vi "query UL_DL Center Channel Number.vi"(8 "error in (no error)":errorcluster, 9 "Direction":T2, 10 "Selected CC Argements":T1, 11 "NR in":refnum<class "NR.lvclass">) -> (0 "error out":errorcluster, 2 "Center Channel Number":u32, 3 "NR out":refnum<class "NR.lvclass">)   [LabVIEW 2023, in "ANRITSU Call Box.lvlib" / "NR.lvclass"]
uses:
  NR.lvclass
  NR.lvclass/NR.ctl
  Type Definition/Uplink Downlink Enum.ctl
  ANRITSU Call Box.lvlib
  Type Definition/NR Selected CC Type Arguments.ctl
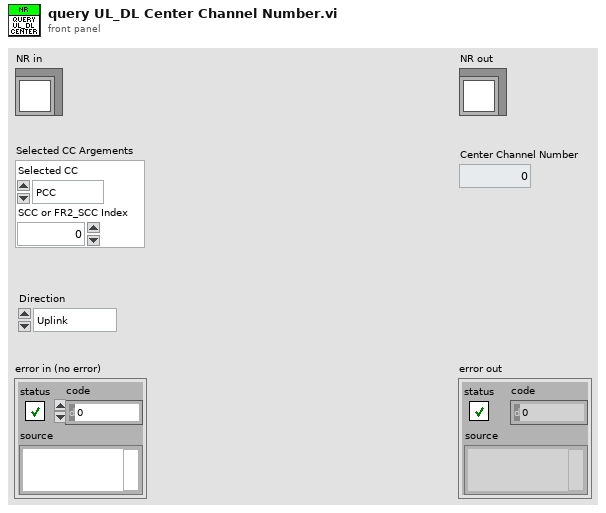
[diagram p1: front panel]
types:
  T1 = typedef "ANRITSU Call Box.lvlib/NR Selected CC Type Arguments.ctl" = cluster{"Selected CC":enum16{"PCC", "SCC", "FR2_PCC", "FR2_SCC"}, "SCC or FR2_SCC Index":u32}
  T2 = typedef "ANRITSU Call Box.lvlib/Uplink Downlink Enum.ctl" = enum16{"Uplink", "Downlink"}
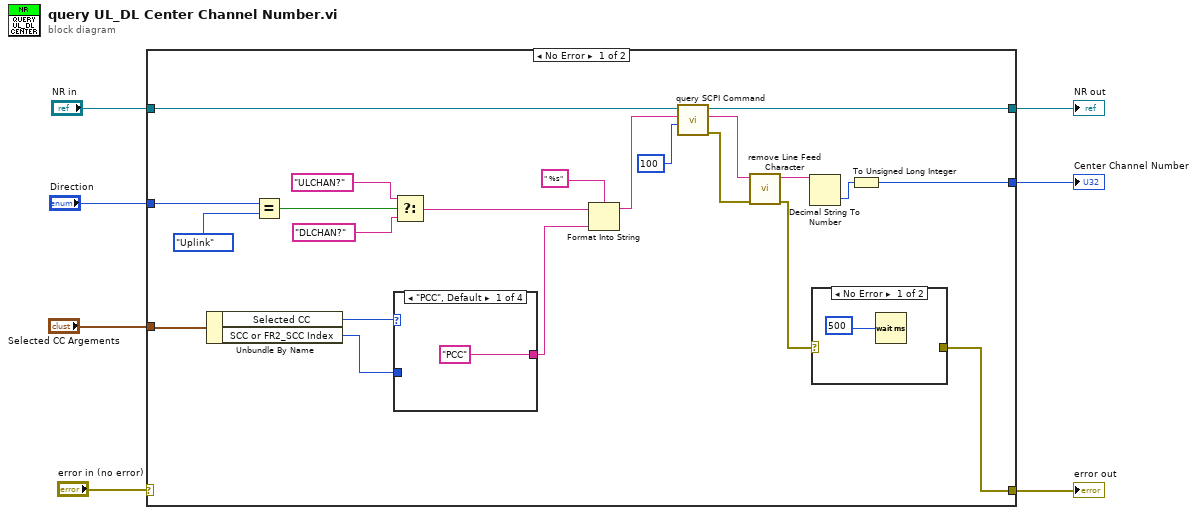
[diagram p0: block diagram]
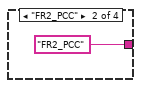
[diagram p3: hidden frame]
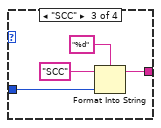
[diagram p4: hidden frame]
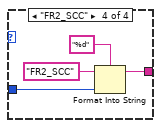
[diagram p5: hidden frame]
diagram:
  n1 = case shown="No Error" "error in (no error)" {
    selector: "error in (no error)" -> [_ w43]
    tunnel: [w20 w43] -> w4
    tunnel: [w14 w42] -> w6
    tunnel: "NR in" -> [w17 w42]
    tunnel: "Selected CC Argements" -> [w21 _]
    tunnel: "Direction" -> [w19 _]
    tunnel: [w8 _] -> w1
    frame No Error {
      n2 = Unbundle By Name(w21) -> ("Selected CC"=w25:enum16{"PCC", "SCC", "FR2_PCC", "FR2_SCC"}, "SCC or FR2_SCC Index"=w24:u32)
      n3 = Equal?(x=w19, y=Uplink_Downlink_Enum."Uplink") -> (x = y?=w26:bool)
      n4 = case shown="\"PCC\", Default" w25 {
        tunnel: ["PCC" "FR2_PCC" w34 w38] -> w22
        tunnel: w24 -> [_ _ w35 w39]
        frame "PCC", Default {
        }
        frame "FR2_PCC" {
        }
        frame "SCC" {
          n5 = Format Into String(format string="%d", initial string="SCC", w35) -> (resulting string=w34:string)  [unwired: 1 in, 1 out]
        }
        frame "FR2_SCC" {
          n6 = Format Into String(format string="%d", initial string="FR2_SCC", w39) -> (resulting string=w38:string)  [unwired: 1 in, 1 out]
        }
      }
      n7 = Select(t="ULCHAN?", s=w26, f="DLCHAN?") -> (s? t:f=w23:string)
      n8 = Format Into String(format string=" %s", initial string=w23, w22) -> (resulting string=w16:string)  [unwired: 1 in, 1 out]
      n9 = call "query SCPI Command.vi"("Read Buffer Length"=u32 100, "SCPI Command"=w16, "NR in"=w17) -> ("error out"=w12:errorcluster, "Read Buffer String"=w13:string, "NR out"=w14:refnum<class "NR.lvclass">)  [unwired: 6 in]
      n10 = call "remove Line Feed Character.vi"("error in"=w12, "Query String"=w13) -> ("error out"=w9:errorcluster, "Line Feed Removed String"=w10:string)  [unwired: 8 in]
      n11 = Decimal String To Number(string=w10) -> (number=w11:i32)  [unwired: 2 in, 1 out]
      n12 = case shown="No Error" w9 {
        selector: w9 -> [_ w31]
        tunnel: [_ w31] -> w20
        frame No Error {
          n13 = Wait (ms)(milliseconds to wait=u32 500) -> ()  [unwired: 1 out]
        }
        frame Error {
        }
      }
      n14 = To Unsigned Long Integer(number=w11) -> (unsigned 32bit integer=w8:u32)
    }
    frame Error {
    }
  }
  "error out" <- w4
  "NR out" <- w6
  "Center Channel Number" <- w1
